vi "OwnCompat20261012_Native_MoveTerminal.vi"() -> ()   [LabVIEW 2024]
panel:
  out "error out":errorcluster caption="错误输出"
  in  "y":i16=100
  in  "x":i16=100
  in  "owner_diagram_id":u32
  in  "terminal_id":u32
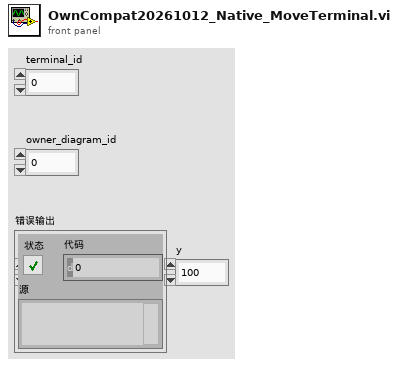
[diagram p1: front panel]
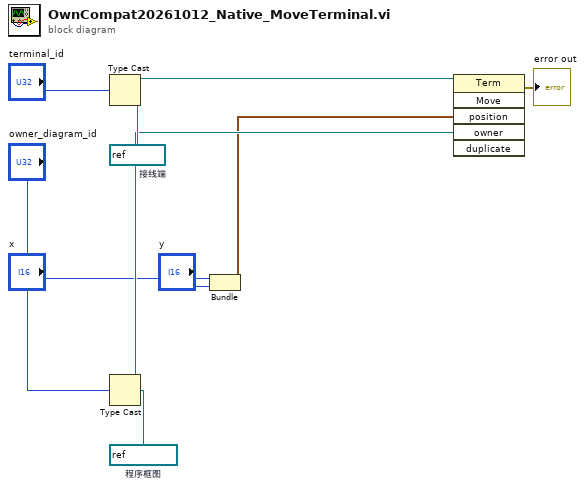
[diagram p0: block diagram]
diagram:
  w7 = refnum<vi> refnum  # 程序框图
  w9 = refnum<vi> refnum  # 接线端
  n1 = Type Cast ("强制类型转换")(type=w9, x="terminal_id") -> (*(type *) &x=w6:refnum<vi>)
  n2 = Type Cast ("强制类型转换")(type=w7, x="owner_diagram_id") -> (*(type *) &x=w5:refnum<vi>)
  n3 = Bundle ("捆绑")("x"="x", "y"="y") -> (w2:cluster{"x":i16, "y":i16})  [unwired: 1 in]
  n4 = invoke class="Term" method="Move"(reference=w6, "position"=w2, "owner"=w5) -> (error out=→"error out":errorcluster)  [unwired: 3 in, 5 out]
